vi "write VISA Command with TermChar.vi"(8 "error in (no error)":errorcluster, 10 "Command String":string, 11 "3D Controller in":refnum<class "3D Controller.lvclass">) -> (0 "error out":errorcluster, 3 "3D Controller out":refnum<class "3D Controller.lvclass">)   [LabVIEW 2023, in "FCC 3D Controller for BS.lvlib" / "3D Controller.lvclass"]
uses:
  3D Controller.lvclass
  3D Controller.lvclass/3D Controller.ctl
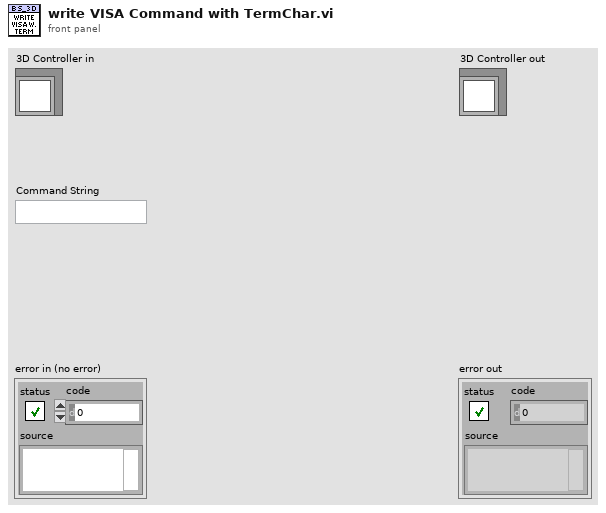
[diagram p1: front panel]
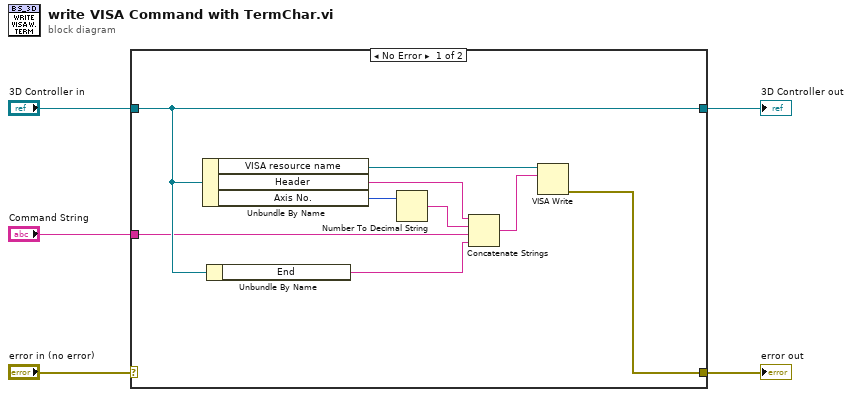
[diagram p0: block diagram]
diagram:
  n1 = case shown="No Error" "error in (no error)" {
    selector: "error in (no error)" -> [_ w16]
    tunnel: [w8 w16] -> w4
    tunnel: [w11 w15] -> w2
    tunnel: "3D Controller in" -> [w11 w15]
    tunnel: "Command String" -> [w10 _]
    frame No Error {
      n2 = Unbundle By Name(w11) -> ("VISA resource name"=w7:refnum<visa-resource-name>, "Header"=w14:string, "Axis No."=w13:i32)
      n3 = Unbundle By Name(w11) -> ("End"=w6:string)
      n4 = Number To Decimal String(number=w13) -> (decimal integer string=w12:string)  [unwired: 1 in]
      n5 = Concatenate Strings(w14, w12, w10, w6) -> (w9:string)
      n6 = VISA Write(VISA resource name=w7, write buffer=w9) -> (error out=w8:errorcluster)  [unwired: 1 in, 2 out]
    }
    frame Error {
    }
  }
  "error out" <- w4
  "3D Controller out" <- w2
